vi "AlliGator Phasor Ratio Graph Panel.vi"() -> ()   [LabVIEW 2021, in "AlliGator Phasor Ratio.lvlib"]
uses:
  AlliGator Phasor Ratio.lvlib
  Phasor/Phasor Ratio Type.ctl
  AlliGator Phasor Ratio Graph Ctrl Refnums.ctl
  Globals, Variables, Constants/AlliGator Refnums List.ctl
  Settings/AlliGator Settings List.ctl
  Graphs/XY Graph/XY Graph Event.ctl
  <vilib>/Utility/miscctls.llb/LVPoint32TypeDef.ctl
  Action Engine/AlliGator Q Element.ctl
  Action Engine/AlliGator Q Event.ctl
  Graphs/XY Graph/XY Graph Mouse Click Event Data.ctl
  Graphs/XY Graph/XY Graph Refnum.ctl
  Graphs/XY Graph/New Plot Information.ctl
  Graphs/Plot Scales.ctl
  Graphs/LabVIEW Plot Interpolation.ctl
  Graphs/Plot Point Style.ctl
  Lifetime & Other Parameters/AlliGator Lifetime & Other Parameters Ctrl Refnums.ctl
  Variant/Variant to Data/Variant to Boolean.vi
  Settings/AlliGator Settings+.lvlib
  Variant/Variant to Data/Variant to Data.lvlib
  Notebook/Notebook.lvlib
  Action Engine/AlliGator Action Engine.lvlib
  GUI/GUI.lvlib
  GUI/AlliGator GUI.lvlib
  Error/Error.lvlib
  Graphs/XY Graph/XY Graph Add-Ons.lvlib
  Python Plugins API/AlliGator Python Plugins.lvlib
  Decay Analysis/Decay Processing/AlliGator Decay Processing.lvlib
  Graphs/Graphs.lvlib
  Lifetime & Other Parameters/AlliGator Lifetime & Other Parameters.lvlib
  Utilities/Utilities.lvlib
  Phasor/Phasor.lvlib
panel:
  in  "Pin Button":bool=TRUE
  out "Phasor Ratio Graph TipStrip":string caption="Lifetime Graph TipStrip"
  out "Phasor Ratio Graph":cluster{"X Array":dbl[], "Y Array":dbl[]}[](graph)
  in  "Phasor Ratio Type":T1
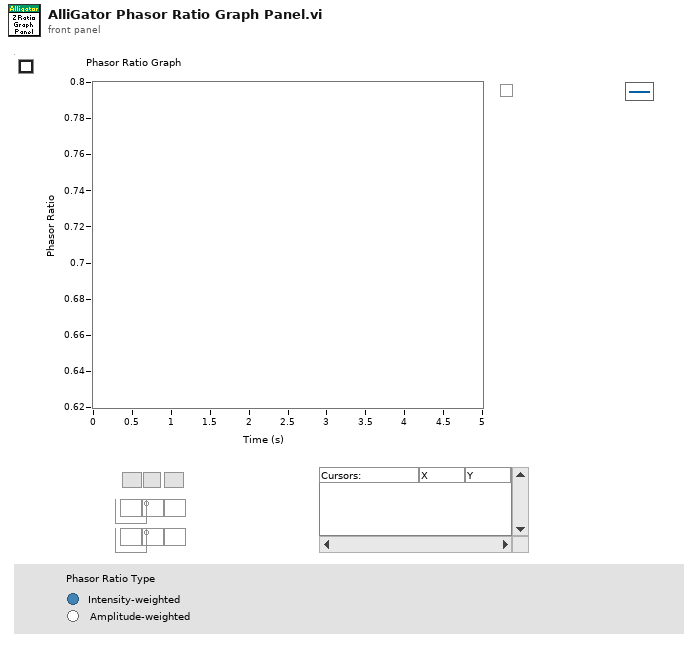
[diagram p1: front panel]
types:
  T1 = typedef "Phasor.lvlib/Phasor Ratio Type.ctl" = enum32{"Intensity-weighted", "Amplitude-weighted"}
  T2 = typedef "AlliGator GUI.lvlib/AlliGator Refnums List.ctl" = enum16{"---------- AlliGator Control Refnums ----------", "AlliGator Tab Control Refnum", "Dataset Ctrl Refnums", "Image Histogram Ctrl Refnums", "Intensity Time Trace Ctrl Refnums", "Decay Graph Ctrl Refnums", "Decay Statistics Graph Ctrl Refnums", "Phasor Graph Ctrl Refnums", "Phasor Ratio Graph Ctrl Refnums", "Phasor Plot Ctrl Refnums", "Lifetime & Other Parameters Ctrl Refnums", "Decay Fit Parameter Map Ctrl Refnums", "Parameter Map Ctrl Refnums", "Other AlliGator Ctrl Refnums", "---------- AlliGator Menu Refnums ----------", "AlliGator Menu", "---------- IO Device ID ----------", "Mouse ID", "Keyboard ID"}
  T3 = typedef "AlliGator Phasor Ratio.lvlib/AlliGator Phasor Ratio Graph Ctrl Refnums.ctl" = cluster{"Phasor Ratio Graph":refnum<vi>}
  T4 = cluster{"Event Registration Refnum":refnum<event-registration>, "Event Registration Refnum":refnum<event-registration>}
  T5 = typedef "AlliGator Settings+.lvlib/AlliGator Settings List.ctl" = enum16{"GUI:Visible Settings Tab", "GUI:Last Run Version", "Source Image:Use Image Histogram for Contrast", "Source Image:Low Count Pixels Rejection Options", "Source Image:High Count Pixels Rejection Options", "Source Image:Use Image Brightness", "Source Image:Blend Overlay with Image Background", "Source Image:Use Fixed ROI Diameter", "Source Image:ROI Diameter", "Source Image:ROI Center Color", "Source Image:Peak Threshold", "Source Image:Intensity Threshold", "Source Image:Image Binning Options", "Source Image:Image Smoothing Options", "Source Image:Image Histogram Active", "Source Image:Invert Binary Mask", "Source Image:Hot Pixel Removal", "Source Image:Overlay Analyzed ROI Center", "Source Image:Auto-Adjust Contrast", "Source Image:Histogram Lower Percentile", "Source Image:Histogram Upper Percentile", "Source Image:Lock ROI with Maps", "Source Image:Save Source Image", "Source Image:Scale Bar Options", "Source Image:Image Resolution (Pixel Size)", "Source Image:Flatfield Correction", "Source Image:Show Dead Left Columns Correction", "Source Image:Dead Left Columns Correction", "Source Image:Image Pre-Processing Operations Order", "Source Image:Overlay ROI Median", "Source Image:Median Overlay Color", "Data Information:Gate Width", "Data Information:Nanotime Gate Separation", "Data Information:Macrotime Gate Separation", "Data Information:Gate Step", "Data Information:# Gates", "Data Information:Gate Image Exposure", "Data Information:Gate Image Integration", "Data Information:Gates to Skip", "Data Information:Gates to Keep", "Data Information:Define Gates to", "Data Information:Channel Name", "Data Information:Available Channel Names", "Data Information:Channel Arithmetic", "Data Information:Background File Subtraction", "Data Information:Background File", "Data Information:Background Scaling Factor", "Data Information:Background Pile-up Correction", "Data Information:Background Pixel Well Capacity", "Data Information:Laser Period", "Data Information:SYNC Period", "Data Information:Pile-up Correction", "Data Information:Pixel Well Capacity", "Data Information:Dataset Scaling Factor", "Fluorescence Decay_Decay Pre-Processing:Reverse Gates", "Fluorescence Decay_Decay Pre-Processing:Verbose Decay Pre-Processing", "Fluorescence Decay_Decay Pre-Processing:Use Decay Pre-Processing", "Fluorescence Decay_Decay Pre-Processing:Background Subtraction", "Fluorescence Decay_Decay Pre-Processing:Background Definition Range", "Fluorescence Decay_Decay Pre-Processing:Baseline Subtraction Method", "Fluorescence Decay_Decay Pre-Processing:Decay Pre-Processing Operations Order", "Fluorescence Decay_Decay Pre-Processing:Smoothing Parameter", "Fluorescence Decay_Decay Pre-Processing:Shift Decay", "Fluorescence Decay_Decay Pre-Processing:Decay Shift Parameters", "Fluorescence Decay_Decay Pre-Processing:Fold Decay", "Fluorescence Decay_Decay Pre-Processing:# Folds", "Fluorescence Decay_Decay Pre-Processing:1-Normalize Decay", "Fluorescence Decay_Decay Pre-Processing:[0-1]-Normalize Decay", "Fluorescence Decay_Decay Pre-Processing:Smoothen Decay", "Fluorescence Decay_Decay Pre-Processing:Extrapolate Decay", "Fluorescence Decay_Decay Pre-Processing:Use Periodicity", "Fluorescence Decay_Decay Pre-Processing:Use Cursors", "Fluorescence Decay_Decay Pre-Processing:Tail Fraction", "Fluorescence Decay_Decay Pre-Processing:Head Fraction", "Fluorescence Decay_Decay Pre-Processing:Additional Points", "Fluorescence Decay_Decay Pre-Processing:Straighten Decay", "Fluorescence Decay_Decay Pre-Processing:Constant Background", "Fluorescence Decay_Decay Pre-Processing:Pixel-Normalize Decay", "Fluorescence Decay_Advanced Analysis:Extract IRF instead of Decay", "Fluorescence Decay_Advanced Analysis:IRF Extraction Options", "Fluorescence Decay_Advanced Analysis:IRF Optimization Options", "Fluorescence Decay_Advanced Analysis:Square Pulse Options", "Fluorescence Decay_Advanced Analysis:IRF Order", "Fluorescence Decay_Advanced Analysis:IRF Time Constants", "Fluorescence Decay_Advanced Analysis:Wavelet Analysis Options", "Fluorescence Decay_Advanced Analysis:Average Lifetime Options", "Fluorescence Decay_Fit Options:Fit Options", "Fluorescence Decay_Fit Options:Use Legacy Fitting Approach", "Fluorescence Decay_Fit Options:Use Data Information Laser Period", "Fluorescence Decay_Fit Parameters:Displayed Fit Parameters", "Fluorescence Decay_Fit Parameters:Fit Parameter Constraints", "Fluorescence Decay_Fit Parameters:Export Tabulated Results", "Fluorescence Decay_Fit Parameters:MLE Baseline Offset Type", "Fluorescence Decay_Fit Parameters:MLE Baseline Offset", "Fluorescence Decay_Fit Parameters:Guess Parameter Names", "Fluorescence Decay_Fit Parameters:Guess Parameter Values", "Fluorescence Decay_Fit Parameters:Guess Parameters Options", "Fluorescence Decay_Fit Parameters:Optimal Offset Selection Criterion", "Fluorescence Decay_Styles:Show Last Decay Only", "Fluorescence Decay_Styles:Decay Graph Color Array", "Fluorescence Decay:Decay Graph Active", "Fluorescence Decay Statistics:Min Peak Value", "Fluorescence Decay Statistics:Reject Low Decay Peak Pixels", "Fluorescence Decay Statistics:Reject High Decay Peak Pixels", "Fluorescence Decay Statistics:Max Peak Value", "Time Traces:Use File Timestamp", "Time Traces:Time Step", "Time Traces:Use Intensity Correction File", "Time Traces:Intensity Correction File", "Phasor Plot:Phasor Plot Smoothing Options", "Phasor Plot:Phasor Plot Size", "Phasor Plot:Phasor Plot Graphics Options", "Phasor Plot:Cumulative Phasor Plot", "Phasor Plot:Use Phasor Brightness", "Phasor Plot:Blend Overlay with Phasor Background", "Phasor Plot:Save Phasor Plot", "Phasor Plot:Show References", "Phasor Plot:Phasor Ratio Decay Range", "Phasor Plot:Exponential Fading", "Phasor Plot:Phasor Ratio Reference Colors", "Phasor Plot:Reference Radius", "Phasor Plot:Show Color Map Vertices", "Phasor Plot:Phasor Plot Active", "Phasor Plot:Phasor Ratio Color Map Type", "Phasor Plot:Phasor Ratio Color Map", "Phasor Plot:Phasor Ratio Display Range", "Phasor Plot:Selected Image ROI(s)", "Phasor Plot:All Image ROIs", "Phasor Plot:Selected Phasor Plot ROI(s)", "Phasor Plot:All Phasor Plot ROIs", "Phasor Plot:Phasor Ratio Color-Coded Quantity", "Phasor Plot:Store Phasor Harmonics", "Phasor Plot:Draw Reference Segment", "Phasor Plot:User-Defined Quantity", "Phasor Plot:Color Scale High Color", "Phasor Plot:Color Scale Low Color", "Phasor Plot:Intensity-weighted Phasor Plot", "Phasor Graph:Phasor Frequency", "Phasor Graph:Phasor Ratio Type", "Phasor Graph:Pixel-level Phasor Computation", "Phasor Graph:Save Phasor Graph", "Phasor Graph:Phasor Graph Active", "Phasor Graph:Phasor SDV Options", "Phasor Graph:Intensity-weighted Phasor Graph", "Phasor Graph:Define Shortest Lifetime as", "Phasor Calibration:Use Backup Calibration if needed", "Phasor Calibration:Backup Calibration Type", "Phasor Calibration:Calibration Type", "Phasor Calibration:Calibration Lifetime", "Phasor Calibration:Calibration Map Algorithm", "Single-Exponential Phasor Locus (SEPL):Gate Parameters", "Single-Exponential Phasor Locus (SEPL):User-defined Gate", "Single-Exponential Phasor Locus (SEPL):User-defined IRF", "Single-Exponential Phasor Locus (SEPL):Phasor Parameters", "Single-Exponential Phasor Locus (SEPL):Decay & IRF Parameters", "Single-Exponential Phasor Locus (SEPL):Display Parameters", "Lifetime Analysis:Decay Analysis Parameters", "Lifetime Analysis:Lifetime Map Active", "Plugins:Python Settings", "Miscellaneous:Verbose Mode", "Miscellaneous:Beep after Script", "Miscellaneous:Saved Image File Format", "Miscellaneous:Exported Gate Image Settings", "Miscellaneous:Include Loading in Timing", "Miscellaneous:Verbose Settings Mode", "Miscellaneous:Histogram Options", "Miscellaneous:Beep on Error", "Miscellaneous:# Logical Processors Used", "Miscellaneous:ROI Description Max Characters", "Miscellaneous:Verbose Error Mode", "Miscellaneous:Transparent Mask Color"}
  T6 = typedef "XY Graph Add-Ons.lvlib/XY Graph Event.ctl" = cluster{"Item Tag":string, "XY Graph Refnum":refnum<vi>, "Coords":T7, "Item Path":string}
  T7 = typedef "LVPoint32TypeDef.ctl" = cluster{"Horizontal":i32, "Vertical":i32}
  T8 = enum16{"0", "1", "2", "3", "4", "5", "6", "7", "8", "9", "A", "B", "C", "D", "E", "F", "G", "H", "I", "J", "K", "L", "M", "N", "O", "P", "Q", "R", "S", "T", "U", "V", "W", "X", "Y", "Z", "F1", "F2", "F3", "F4", "F5", "F6", "F7", "F8", "F9", "F10", "F11", "F12", "F13", "F14", "F15", "ADD", "BACK", "BACKSLASH", "CAPITAL", "COMMA", "DECIMAL", "DELETE", "DIVIDE", "DOWN", "END", "EQUALS", "ESCAPE", "GRAVE (`)", "HOME", "INSERT", "LBRACKET", "LCONTROL", "LEFT", "L ALT", "LSHIFT", "LWIN", "MINUS", "MULTIPLY", "NEXT", "NUMLOCK", "NUMPAD_0", "NUMPAD_1", "NUMPAD_2", "NUMPAD_3", "NUMPAD_4", "NUMPAD_5", "NUMPAD_6", "NUMPAD_7", "NUMPAD_8", "NUMPAD_9", "PAUSE", "PERIOD", "PRIOR (PG UP)", "RBRACKET", "RCONTROL", "RETURN", "RIGHT", "R ALT", "RSHIFT", "RWIN", "SCROLL", "SEMICOLON", "SLASH", "SPACE", "SUBTRACT", "TAB", "UP", "ENTER (num pad)", "' (quote)"}
  T9 = typedef "AlliGator Action Engine.lvlib/AlliGator Q Element.ctl" = cluster{"AlliGator Q Event":T10, "Data":variant}
  T10 = typedef "AlliGator Action Engine.lvlib/AlliGator Q Event.ctl" = enum16{"---- Files ----", "Files:Set Batch Export Files To Save", "Files:Set Dataset Loading & Pre-processing Options", "Files:Check #Frames in Dataset", "Files:Increment Frame Index", "Files:Open Mask Image", "Files:Open White Light Image", "Files:Open Single Dataset", "Files:New Folder of Folders Selected", "Files:Load File (all Types)_Scriptable", "Files:Move Flattened Series to Folders Series", "Files:Select Folder", "Files:Load FLI Dataset", "Files:Load Swiss SPAD 1 Dataset", "Files:Load Swiss SPAD 2 Dataset", "Files:Load .sdt FLI Dataset", "Files:Load .ptu FLI Dataset", "Files:Load .bin FLI Dataset", "Files:Load Single Gate Image Folder", "Files:Load I/m/phi Dataset (deprecated)", "Files:Load Single Image", "Files:Subtract Background File", "Files:Export FLI Dataset", "Files:Load HDF5 FLI Dataset", "Files:Set Destination File Path", "Files:Save Mask Image", "Files:Batch Conversion", "Files:New Folder Selected", "Files:Close FLI Dataset", "Files:Close FLI Dataset Series", "Files:Close White Light Image", "Files:Close Mask Image", "---- FLI Dataset ----", "FLI Dataset:Channel Arithmetic", "FLI Dataset:Export Average Lifetime Map as ASCII", "FLI Dataset:Export User-Defined Quantity Map as ASCII", "FLI Dataset:Python Function FLI Dataset Event", "FLI Dataset:ROI Analysis", "FLI Dataset:Tilted Logistic Square Gated IRF Characteristics Map", "FLI Dataset:Logistic Square Gated IRF Characteristics Map", "FLI Dataset:Square Gated IRF Characteristics Map", "FLI Dataset:Multi-ROI Single-Pixel Phasor Analysis", "FLI Dataset:Multi-ROI Single-Pixel NLSF Analysis", "FLI Dataset:All ROIs IRF Extraction", "FLI Dataset:All ROIs Decay Fit Non-Interactive (Fast + Individual IRF)", "FLI Dataset:All ROIs Phasor Analysis", "FLI Dataset:All ROIs Decay Fit", "FLI Dataset:Fluorescence Decay Statistics", "FLI Dataset:Update Decay Statistics Graph", "FLI Dataset:Get Decay from ROI", "FLI Dataset:All ROIs Average Lifetimes", "FLI Dataset:Save/Load Local IRFs", "FLI Dataset:Clear Local IRFs", "FLI Dataset:Phasor Calibration Maps (# Gates Series) Script", "FLI Dataset:Calibrated Phasor Map Series", "---- FLI Dataset Series ----", "FLI Dataset Series:Sum All Datasets in Series", "FLI Dataset Series:Add Dataset to Accumulated Dataset", "FLI Dataset Series:Display Accumulated Dataset", "FLI Dataset Series:Clear Dataset Series Sum", "FLI Dataset Series:Time-Series Analysis (NLSF)", "FLI Dataset Series:Time-Series Analysis (Phasor)", "---- Image ----", "Image:Update Image Profile Plots", "Image:Image Histogram Cursor Move", "Image:Image Histogram", "Image:Image Contrast", "Image:Set Image Histogram Cursor Move Flag", "Image:Clear Image Overlay", "Image:Use ROI as Search Area", "Image:Set ROI Diameter", "Image:Save Image Data as TIFF", "Image:Save Displayed Image with Overlay", "Image:Save Image Overlay Only", "Image:Save Image as Hot Pixel Mask", "Image:Change Source Image Color Palette", "Image:Copy Image to Clipboard", "Image:Source Image ROI Selection", "Image:Delete All ROIs", "Image:Delete All Unselected ROIs", "Image:Delete ROI", "Image:Merge All ROIs", "Image:Store ROI", "Image:Source Image ROI Storage", "Image:Export ROI Description to Notebook", "Image:Save ROI", "Image:Load ROI", "Image:Paste ROI Definition", "Image:Clear ROI", "Image:Identify ROIs in Mask Image", "Image:Create Complementary ROI", "Image:Create Contour ROI", "Image:Create ROI(s) from Pixels with Peak above Min_Scriptable", "Image:Create ROI(s) from Pixels with Intensity above Min_Scriptable", "Image:Compute ROI Statistics", "Image:Delete ROI(s) based on ROI Characteristics", "Image:Create ROI Grid", "Image:ROI to Individual Pixel ROIs", "Image:Python Function Source Image Event", "Image:Show Phasor Calibration Map ROI Centers", "Image:Convert ROI to Mask Image", "Image:Mouse Move", "Image:Mouse Up", "Image:Set Source Image Mouse Move Flag", "Image:Add Scale Bar Overlay", "Image:Delete Existing ROIs Option", "Image:Overlay ROI Median", "Image:Check Current ROI", "Image:Update True Pixel Value", "Image:Use ROI", "---- Decay ----", "Decay:Clear IRF/Reference Plot", "Decay:Add Decay to Graph", "Decay:Smoothen Plot", "Decay:Smoothen Plot Tail", "Decay:Average Selected Plots", "Decay:Extract IRF", "Decay:Optimal IRF Extraction", "Decay:Threshold IRF", "Decay:Fit to Model IRF", "Decay:Fit IRF to Square Gate", "Decay:Fit IRF to Logistic Square Gate", "Decay:Fit IRF to Tilted Logistic Square Gate", "Decay:Create Bounding Cursors Set", "Decay:Export Bounding Cursors Definition to Notebook", "Decay:Denoise Plot", "Decay:Compute Cumulative Function", "Decay:Use as Reference Decay", "Decay:Show Reference Decay/IRF", "Decay:Extrapolate Decay", "Decay:Create Head & Tail Bounding Cursors", "Decay:Store Cursor-defined Head & Tail Fractions", "Decay:Rebin Plot", "Decay:1-Normalize Decay", "Decay:[0-1]-Normalize Plot", "Decay:Straighten Decay", "Decay:Shift Decay", "Decay:Fold Decay", "Decay:Fit Decay", "Decay:Global Fit of Selected Decays", "Decay:Post Global Fit Script", "Decay:Add Global Fit Parameters to Graph", "Decay:Add Decay Parameter(s) to Plot (Graph)", "Decay:Export Decay to Phasor Graph", "Decay:Compute Average Lifetime", "Decay:Plot Convolution", "Decay:Graph Tip Strip Update", "---- Decay Statistics ----", "Decay Statistics:Tip Strip Update", "---- Intensity Time Trace ----", "Intensity Time Trace:Use File Timestamp", "Intensity Time Trace:Load Intensity Corrections File", "Intensity Time Trace:Clear Intensity Corrections File", "Intensity Time Trace:Tip Strip Update", "---- Phasor Plot ----", "Phasor Plot:Build Phasor Plot", "Phasor Plot:Change Phasor Plot Color Palette", "Phasor Plot:Adjust Phasor Plot Display Range", "Phasor Plot:Highlight Image ROI in Phasor Plot", "Phasor Plot:Save Phasor Plot Image with Overlay", "Phasor Plot:Export Complex Phasor Map", "Phasor Plot:Export Phasor Ratio Map", "Phasor Plot:Export Average Lifetime Map", "Phasor Plot:Compute Phase Lifetime Histogram", "Phasor Plot:Compute Phasor Ratio Histogram", "Phasor Plot:Compute Phase Lifetime vs Intensity Scatter Plot", "Phasor Plot:Weber 2-Component Decomposition", "Phasor Plot:Update Phasor Color Map Vertices", "Phasor Plot:Clear Phasor Overlay", "Phasor Plot:Use Segment Extremities as References", "Phasor Plot:Use UC/Segment Intersections as References", "Phasor Plot:Use UC/Principal Axis Intersections as References", "Phasor Plot:Use UC/Linear Fit Intersections as References", "Phasor Plot:Update Phasor Plot Reference", "Phasor Plot:Show Local Phasor Info in Phasor Plot", "Phasor Plot:Update Phasor Plot State", "Phasor Plot:Phasor Plot ROI Storage", "Phasor Plot:Phasor Plot ROI Selection", "Phasor Plot:Python Function Phasor Plot Event", "Phasor Plot:Overlay Phasor ROI, Ratio or Map in Source Image", "Phasor Plot:Compute Decay of Selected Phasors", "Phasor Plot:Phasor at Image Pixel", "Phasor Plot:Mouse Move", "Phasor Plot:Mouse Up", "Phasor Plot:Display Range Mouse Move", "Phasor Plot:Set Mouse Move Flag", "Phasor Plot:Update True Phasor Plot Value", "---- Phasor Graph ----", "Phasor Graph:Get Phasor Value", "Phasor Graph:Create New Phasor Plot Dialog", "Phasor Graph:Update Last Phasor Value", "Phasor Graph:Update Phasor (m, phi)", "Phasor Graph:Remove Single Phasor from Plot", "Phasor Graph:Add Single Phasor to Plot", "Phasor Graph:Remove Phasor Plot", "Phasor Graph:Remove Selected Phasor Plots", "Phasor Graph:Clear Phasor Data", "Phasor Graph:Clear Phasor Graph", "Phasor Graph:Cursor Move", "Phasor Graph:Draw Cursor Connecting Line", "Phasor Graph:Clear Cursor Connecting Line", "Phasor Graph:Find UC Intersection", "Phasor Graph:Use UC/Cursor-Defined Line Intersections", "Phasor Graph:Use Selected Plots Fitted Line/UC Intersections", "Phasor Graph:Use Selected Plots Principal Axis/UC Intersections", "Phasor Graph:Show Single Phasor", "Phasor Graph:Save Single Phasor Plot", "Phasor Graph:Save All Phasor Plots", "Phasor Graph:Load Phasor Plot(s)", "Phasor Graph:Phasor Multiplication", "Phasor Graph:Compute Average Phasor", "Phasor Graph:Compute Multiple Average Phasors (Selected Plots)", "Phasor Graph:Export Single Phasor Plot Phase Lifetimes", "Phasor Graph:Parameter 2 vs Parameter 1 Scatter Plot", "Phasor Graph:Use Cursor n Location", "Phasor Graph:Set Reference n to Current Phase Lifetime Value", "Phasor Graph:Set Reference n to Lifetime Value", "Phasor Graph:Set Cursor n Location", "Phasor Graph:Save Phasor Graph Image", "Phasor Graph:Update SEPL Plot", "Phasor Graph:Export Single Phasor Plot Data", "Phasor Graph:Export Selected Phasor Plots Data", "Phasor Graph:Python Function Phasor Graph Event", "Phasor Graph:Tip Strip Update", "---- Calibration ----", "Calibration:Set Calibration Type", "Calibration:Load/Save Phasor Calibration", "Calibration:Load/Save Phasor Calibration Series", "Calibration:Load/Save Phasor Calibration Map", "Calibration:Use as Calibration", "Calibration:Compute Optimal Calibration from Phasor References", "Calibration:Clear Phasor Calibration", "Calibration:Single Phasor Calibration Information", "Calibration:Use as Calibration Series", "Calibration:Use as Calibration Map", "Calibration:Clear Calibration Series", "Calibration:Phasor Calibration Series Information", "Calibration:Clear Calibration Map", "Calibration:Phasor Calibration Map Information", "Calibration:Apply Phasor Calibration", "Calibration:Update Single Plot Calibration", "Calibration:Update Multiple Plots Calibration", "Calibration:Clear Single Plot Calibration", "Calibration:Clear All Plots Calibrations", "Calibration:Clear Plot(s) Calibration(s)?", "---- Phasor Ratio ----", "Phasor Ratio:Clear Reference n", "Phasor Ratio:Toggle Selected Plot(s)  Lock to Reference 1", "Phasor Ratio:Use as Reference n", "Phasor Ratio:Send Reference n to Notebook", "Phasor Ratio:Toggle Selected Plot(s)  Lock to Reference 2", "Phasor Ratio:Compute Phasor Ratio at Mouse Location", "Phasor Ratio:Compute Phasor Plot's Average Phasor Ratio", "Phasor Ratio:Compute Time-Series Phasor Ratios", "Phasor Ratio:Fit Line to Phasor Ratio Plot", "Phasor Ratio:Save References", "Phasor Ratio:Load References", "Phasor Ratio:Update Phasor Reference 1", "Phasor Ratio:Update Phasor Reference 2", "Phasor Ratio:Move Cursor n to Reference n", "Phasor Ratio:Use as Phasor Reference 1 Lifetime", "Phasor Ratio:Use as Phasor Reference 2 Lifetime", "Phasor Ratio:Export Phasor Ratio Map as ASCII", "Phasor Ratio:Tip Strip Update", "---- Lifetime & Other Parameters Graph ----", "Lifetime:Compute Sliced Mean, SDV and CV Plots", "Lifetime:Plot Decay Shifts", "Lifetime:Plot Histogram", "---- Decay Fit Parameter Map ----", "Decay Fit Parameter Map:Export ROI NLSF Data as ASCII", "Decay Fit Parameter Map:Set Decay Fit Parameter Map Selection", "Decay Fit Parameter Map:Build Decay Fit Parameter Map", "Decay Fit Parameter Map:Change Decay Fit Parameter Map Color Palette", "Decay Fit Parameter Map:Export Decay Fit Parameter Map Data as ASCII", "Decay Fit Parameter Map:Export All Decay Fit Parameter Maps Data as ASCII", "Decay Fit Parameter Map:Selected Parameter Scatterplot", "Decay Fit Parameter Map:Parameter 2 vs Parameter 1 Scatterplot", "Decay Fit Parameter Map:Save Decay Fit Parameter Map Image", "Decay Fit Parameter Map:Save-Load IRFs & Fit Data", "Decay Fit Parameter Map:Update Local Decay Plots", "Decay Fit Parameter Map:Python Function Decay Fit Parameters Map Event", "Decay Fit Parameter Map:Overlay Decay Fit Parameter Map in Source Image", "Decay Fit Parameter Map:Selected Parameter vs Intensity Scatterplot", "Decay Fit Parameter Map:Mouse Up", "Decay Fit Parameter Map:Mouse Move", "Decay Fit Parameter Map:Display Range Mouse Move", "Decay Fit Parameter Map:Change Map Resolution", "Decay Fit Parameter Map:Variance Significance Maps", "Decay Fit Parameter Map:Fit Result Constraints Window", "Decay Fit Parameter Map:Use ROI", "---- Parameter Map ----", "Parameter Map:Export ROI Parameters Data as ASCII", "Parameter Map:Add Parameter Map Set", "Parameter Map:Delete Parameter Map Set", "Parameter Map:Update Parameter List", "Parameter Map:Build Parameter Map", "Parameter Map:Change Parameter Map Color Palette", "Parameter Map:Export Parameter Map Data as ASCII", "Parameter Map:Export All Parameter Maps Data as ASCII", "Parameter Map:Selected Parameter Scatterplot", "Parameter Map:Parameter 2 vs Parameter 1 Scatterplot", "Parameter Map:Selected Parameter vs Intensity Scatterplot", "Parameter Map:Save Parameter Map Image", "Parameter Map:Save-Load IRFs & Parameter Maps (TODO)", "Parameter Map:Set Parameter Map Selection", "Parameter Map:Python Function Parameter Map Event", "Parameter Map:Overlay Parameter Map in Source Image", "Parameter Map:Update Local Decay Plots", "Parameter Map:Mouse Up", "Parameter Map:Mouse Move", "Parameter Map:Display Range Mouse Move", "Parameter Map:Use ROI", "---- Generic Graph ----", "Generic Graph:Generic XY Graph Event", "Generic Graph:Python Function XY Graph Event", "Generic Graph:New Plot", "Generic Graph:Save Plot", "Generic Graph:XY Plot Histogram", "Generic Graph:Set XY Graph Plot Name", "Generic Graph:Set Last Cursor Style", "Generic Graph:Tip Strip Update", "---- GUI ----", "GUI:Start Script", "GUI:Type of Displayed Image Changed", "GUI:Gate Image Slide Changed", "GUI:Show Busy Icon", "GUI:Show Busy Icon & Abort Button", "GUI:Hide Busy Icon", "GUI:Hide Busy Icon & Abort Button", "GUI:Abort", "GUI:End Script", "GUI:Start Timing", "GUI:End Timing", "GUI:Set State Indicator", "GUI:Send Parameters JSON Strings to Clipboard", "GUI:Set Gate Step", "GUI:Idle", "GUI:Initialization", "GUI:Quit", "GUI:Increment Dataset Index", "GUI:Set Dataset Index to -1", "GUI:Time Series Slider Moved", "GUI:Time Series Slider Changed", "GUI:Toggle Playback or Loop", "GUI:Playback Script", "GUI:Set Phasor Frequency", "GUI:Open Window", "GUI:Start Test Script", "GUI:End Test Script", "GUI:Set Verbose Mode", "GUI:Set Verbose Settings Mode", "GUI:Initialize Python Session", "DEBUG"}
  T11 = typedef "XY Graph Add-Ons.lvlib/XY Graph Mouse Click Event Data.ctl" = cluster{"Multiplot XY Graph":T12, "Mouse Coordinates":T7}
  T12 = typedef "XY Graph Add-Ons.lvlib/XY Graph Refnum.ctl" = refnum<vi>
  T13 = typedef "AlliGator Lifetime & Other Parameters.lvlib/AlliGator Lifetime & Other Parameters Ctrl Refnums.ctl" = cluster{"Lifetime Graph":refnum<vi>}
  T14 = enum16{"0", "1", "2", "3", "4", "5", "6", "7", "8", "9", "A", "B", "C", "D", "E", "F", "G", "H", "I", "J", "K", "L", "M", "N", "O", "P", "Q", "R", "S", "T", "U", "V", "W", "X", "Y", "Z", "F1", "F2", "F3", "F4", "F5", "F6", "F7", "F8", "F9", "F10", "F11", "F12", "F13", "F14", "F15", "ADD", "BACK", "BACKSLASH", "CAPITAL", "COMMA", "DECIMAL", "DELETE", "DIVIDE", "DOWN", "END", "EQUALS", "ESCAPE", "GRAVE (`)", "HOME", "INSERT", "LBRACKET", "LCONTROL", "LEFT", "L ALT", "LSHIFT", "LWIN", "MINUS", "MULTIPLY", "NEXT", "NUMLOCK", "NUMPAD_0", "NUMPAD_1", "NUMPAD_2", "NUMPAD_3", "NUMPAD_4", "NUMPAD_5", "NUMPAD_6", "NUMPAD_7", "NUMPAD_8", "NUMPAD_9", "PAUSE", "PERIOD", "PRIOR (PG UP)", "RBRACKET", "RCONTROL", "RETURN", "RIGHT", "R ALT", "RSHIFT", "RWIN", "SCROLL", "SEMICOLON", "SLASH", "SPACE", "SUBTRACT", "TAB", "UP", "ENTER (num pad)", "' (quote)"}[]
  T15 = typedef "XY Graph Add-Ons.lvlib/New Plot Information.ctl" = cluster{"Multiplot XY Graph":refnum<vi>, "Plot Name":string, "Plot Scales":T16, "Plot Interpolation":T17, "Point Style":T18, "Plot Color":u32, "Plot Metadata":variant}
  T16 = typedef "XY Graph Add-Ons.lvlib/Plot Scales.ctl" = cluster{"X Scale":u32, "Y Scale":u32}
  T17 = typedef "Graphs.lvlib/LabVIEW Plot Interpolation.ctl" = enum16{"Point (.)", "Stepwise Right (--.)", "Line + Point (\\. /)", "Stepwise Left (.--)", "Stepwise Centered (-.-)", "Stepwise Vertical (|.|)", "Line (-)", "Use Previous Plot's Style"}
  T18 = typedef "Graphs.lvlib/Plot Point Style.ctl" = enum16{"not defined", "None", "Empty Circle", "Filled Circle", "Thick Circle", "Dotted Circle", "Empty Square", "Filled Square", "Thick Square", "Dotted Square", "Small Filled Square", "Dot", "Cross", "Tiny Cross", "Large X", "Small x", "Diamond", "Small Empty Square"}
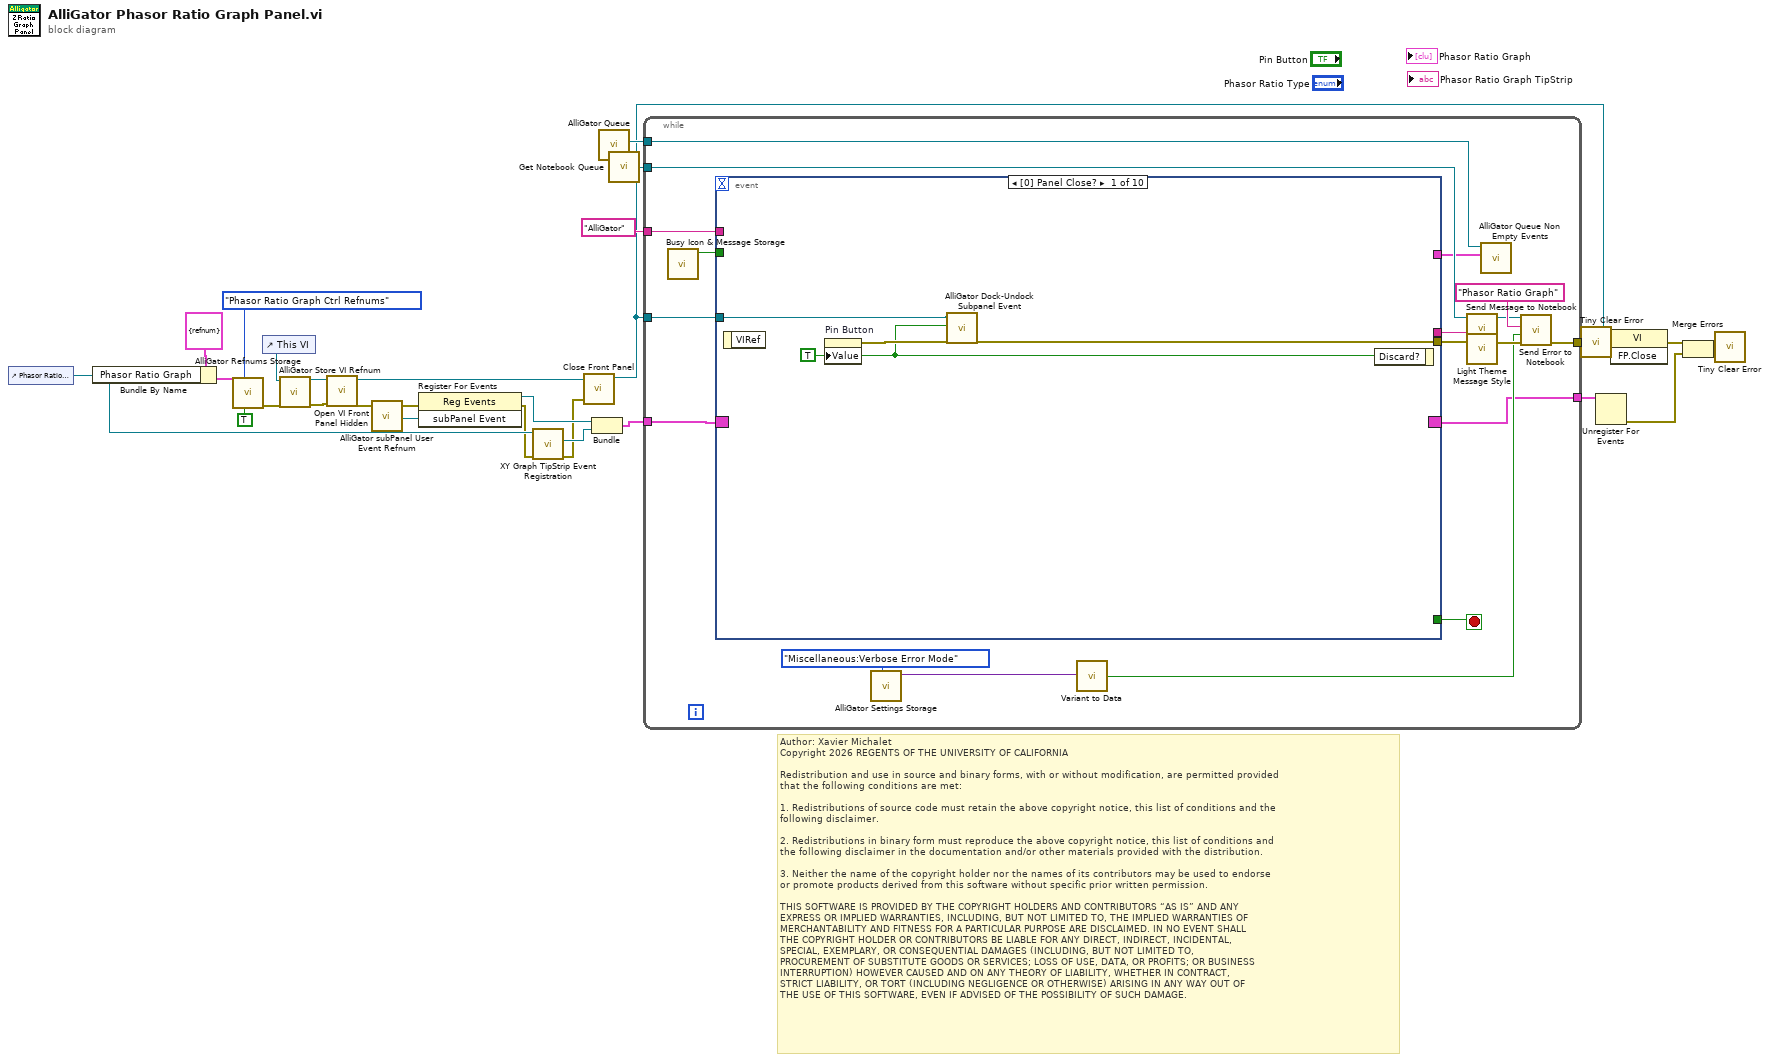
[diagram p0: block diagram]
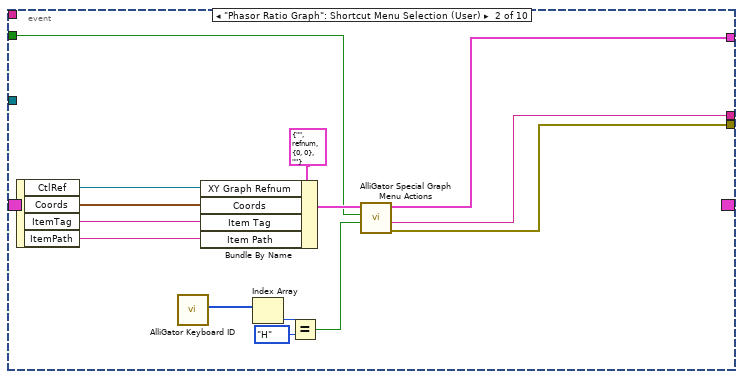
[diagram p2: hidden frame]
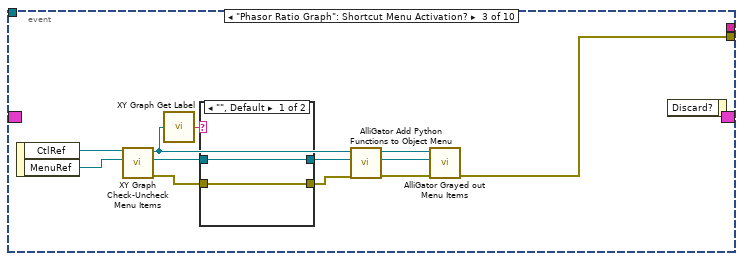
[diagram p3: hidden frame]
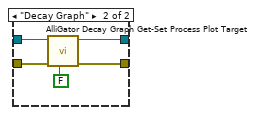
[diagram p4: hidden frame]
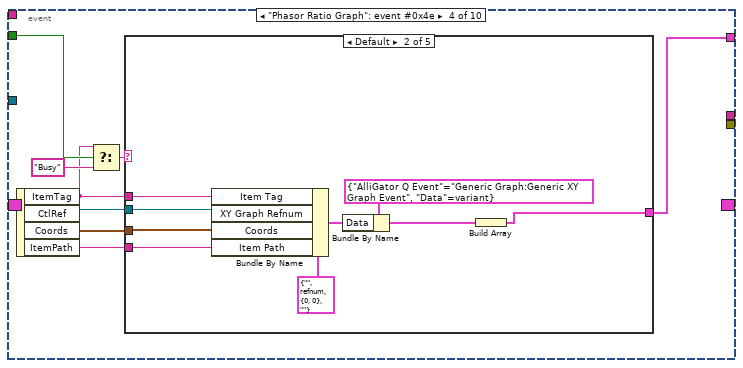
[diagram p5: hidden frame]
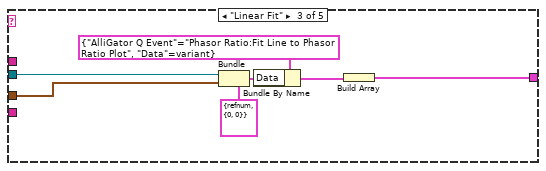
[diagram p7: hidden frame]
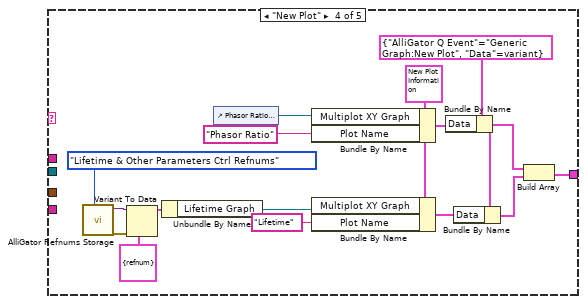
[diagram p8: hidden frame]
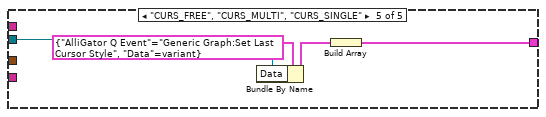
[diagram p9: hidden frame]
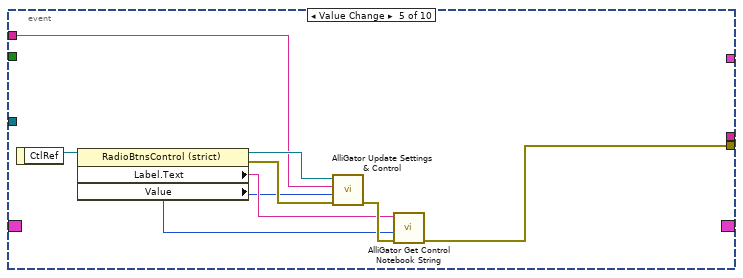
[diagram p10: hidden frame]
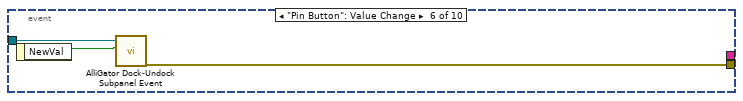
[diagram p11: hidden frame]
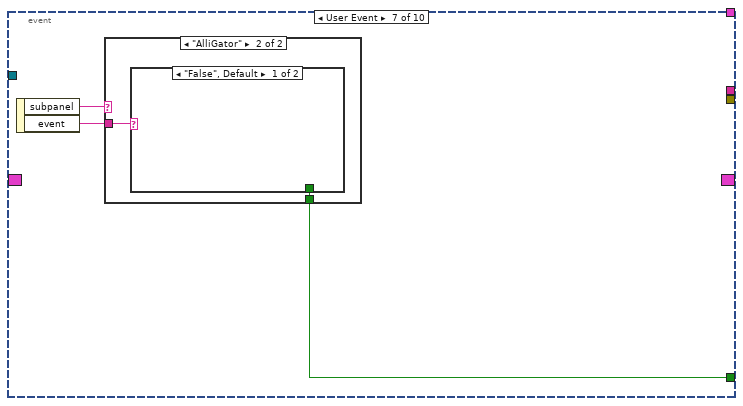
[diagram p12: hidden frame]
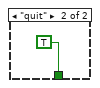
[diagram p14: hidden frame]
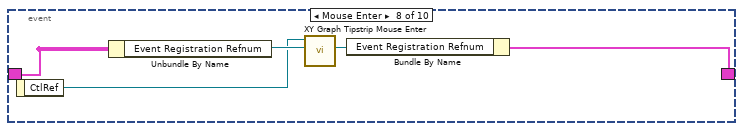
[diagram p15: hidden frame]
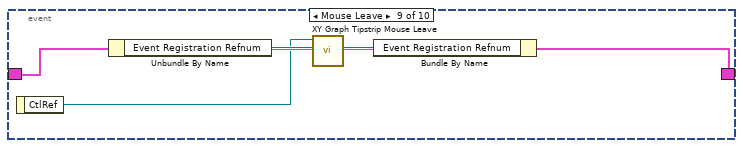
[diagram p16: hidden frame]
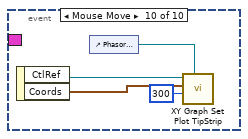
[diagram p17: hidden frame]
diagram:
  # "Author: Xavier Michalet\nCopyright 2026 REGENTS OF THE UNIVERSITY OF CALIFORNIA\n\nRedistribution and use in source and binary forms, with or without modification, are permitted provided\nthat the following conditions are met:\n\n1. Redistributions of source code must retain the above copyright notice, this list of conditions and the\nfollowing disclaimer.\n\n2. Redistributions in binary form must reproduce the above copyright notice, this list of conditions and\nthe following disclaimer in the documentation and/or other materials provided with the distribution.\n\n3. Neither the name of the copyright holder nor the names of its contributors may be used to endorse \nor promote products derived from this software without specific prior written permission.\n\nTHIS SOFTWARE IS PROVIDED BY THE COPYRIGHT HOLDERS AND CONTRIBUTORS “AS IS” AND ANY \nEXPRESS OR IMPLIED WARRANTIES, INCLUDING, BUT NOT LIMITED TO, THE IMPLIED WARRANTIES OF\nMERCHANTABILITY AND FITNESS FOR A PARTICULAR PURPOSE ARE DISCLAIMED. IN NO EVENT SHALL\nTHE COPYRIGHT HOLDER OR CONTRIBUTORS BE LIABLE FOR ANY DIRECT, INDIRECT, INCIDENTAL, \nSPECIAL, EXEMPLARY, OR CONSEQUENTIAL DAMAGES (INCLUDING, BUT NOT LIMITED TO, \nPROCUREMENT OF SUBSTITUTE GOODS OR SERVICES; LOSS OF USE, DATA, OR PROFITS; OR BUSINESS\nINTERRUPTION) HOWEVER CAUSED AND ON ANY THEORY OF LIABILITY, WHETHER IN CONTRACT, \nSTRICT LIABILITY, OR TORT (INCLUDING NEGLIGENCE OR OTHERWISE) ARISING IN ANY WAY OUT OF\nTHE USE OF THIS SOFTWARE, EVEN IF ADVISED OF THE POSSIBILITY OF SUCH DAMAGE."
  n1 = control-ref of="Phasor Ratio Graph"() -> (w15:refnum<vi>)
  n2 = Bundle By Name(cluster=T3 {"Phasor Ratio Graph"=refnum} ("Phasor Ratio Graph Ctrl Refnums"), "Phasor Ratio Graph"=w15) -> (w16:T3)
  n3 = call "AlliGator Refnums Storage.vi"("Get(F)/Set"=TRUE, "AlliGator Refnum List"=AlliGator_Refnums_List."Phasor Ratio Graph Ctrl Refnums", "Data in"=w16) -> ("Error Out"=w4:errorcluster)  [unwired: 7 in, 1 out]
  n4 = control-ref of="This VI"() -> (w1:refnum<vi>)
  n5 = call "AlliGator Store VI Refnum.vi"("error in (no error)"=w4, "VI Refnum"=w1) -> ("error out"=w3:errorcluster, "VI Refnum (dup)"=w2:refnum<vi>)  [unwired: 7 in, 1 out]
  n6 = call "Open VI Front Panel Hidden.vi"("error in"=w3, "VI in"=w2) -> ("error out"=w9:errorcluster, "VI out"=w7:refnum<vi>)  [unwired: 8 in]
  n7 = call "AlliGator subPanel User Event Refnum.vi"() -> ("subPanel Event"=w24:refnum<user-event>)  [unwired: 9 in]
  n8 = register-events(error in=w9, w24) -> (reference out=w23:refnum<event-registration>, error out=w8:errorcluster)  [unwired: 1 in]
  n9 = call "XY Graph TipStrip Event Registration.vi"("error in (no error)"=w8, "XY Graph Refnum"=w15) -> ("error out"=w6:errorcluster, "Event Registration Refnum"=w13:refnum<event-registration>)  [unwired: 7 in, 1 out]
  n10 = call "Close Front Panel.vi"("error in (no error)"=w6, "VI in"=w7) -> ("VI out"=w5:refnum<vi>)  [unwired: 8 in, 1 out]
  n11 = Bundle("Event Registration Refnum"=w23, "Event Registration Refnum"=w13) -> (w14:T4)  [unwired: 1 in]
  n12 = call "AlliGator Queue.vi"() -> ("AlliGator Q"=w26:refnum<queue>)  [unwired: 8 in, 1 out]
  n13 = call "Get Notebook Queue.vi"() -> ("Notebook Queue"=w27:refnum<queue>)  [unwired: 9 in]
  n14 = while {
    tunnel: w27 -> [w38]
    tunnel: w26 -> [w35]
    tunnel: "AlliGator" ("Sender") -> [w33]
    tunnel: w5 -> [w31]
    tunnel: w14 -> [w30]
    tunnel: [w29] -> w22
    tunnel: [w28] -> w21
    stop <- w45 stop-if-true
    n15 = call "Busy Icon & Message Storage.vi"() -> ("Busy Icon Status (F = busy)"=w32:bool)  [unwired: 9 in, 2 out]
    n16 = event shown="[0] Panel Close?" {
      selector: w30 -> [_ _ _ _ _ _ _ w146 w151 _]
      dyn-events: [_ _ _ _ _ _ _ w144 w149 _] -> w29
      timeout: _ -> [_ _ _ _ _ _ _ _ _ _]
      tunnel: [w48 w50 w64 _ w127 w135 _ _ _ _] -> w39
      tunnel: [_ _ _ _ _ _ w138 _ _ _] -> w45
      tunnel: [_ w51 _ _ _ _ _ _ _ _] -> w36
      tunnel: [_ w52 _ w89 _ _ _ _ _ _] -> w34
      tunnel: w32 -> [_ w57 _ w88 _ _ _ _ _ _]
      tunnel: w33 -> [_ _ _ _ w130 _ _ _ _ _]
      tunnel: w31 -> [w47 _ _ _ _ w137 _ _ _ _]
      event Panel Close? {
        w46 = TRUE ("Pin Button")
        n17 = event-data() -> ()  [unwired: 1 in, 1 out]
        n18 = property on="Pin Button" class="Bool (strict)"("Value"=w46) -> (error out=w49:errorcluster)  [unwired: 2 in, 1 out]
        n19 = call "AlliGator Dock-Undock Subpanel Event.vi"("Error In"=w49, "Dock?"=w46, "VI in"=w47) -> ("Error Out"=w48:errorcluster)  [unwired: 8 in]
        n20 = event-data("Discard?"=w46) -> ()  [unwired: 1 in, 1 out]
      }
      event "Phasor Ratio Graph": Shortcut Menu Selection (User) {
        n21 = event-data() -> ("CtlRef"=w53:refnum<vi>, "Coords"=w56:T7, "ItemTag"=w54:string, "ItemPath"=w55:string)  [unwired: 1 in]
        n22 = call "AlliGator Keyboard ID.vi"() -> ("keys pressed"=w63:T14)  [unwired: 9 in, 2 out]
        n23 = Bundle By Name(cluster=T6 {"Item Tag"="", "XY Graph Refnum"=refnum, "Coords"={"Horizontal"=0, "Vertical"=0}, "Item Path"=""} ("XY Graph Event"), "XY Graph Refnum"=w53, "Coords"=w56, "Item Tag"=w54, "Item Path"=w55) -> (w61:T6)
        n24 = Index Array(array=w63) -> (element=w58:T8)  [unwired: 1 in]
        n25 = Equal?(x=w58, y=T8."H" ("element")) -> (x = y?=w62:bool)
        n26 = call "AlliGator Special Graph Menu Actions.vi"("Help?"=w62, "Animated Busy Icon"=w57, "XY Graph Event"=w61) -> ("Error Out"=w50:errorcluster, "Message"=w51:string, "AlliGator Actions"=w52:T9[])  [unwired: 6 in]
      }
      event "Phasor Ratio Graph": Shortcut Menu Activation? {
        n27 = event-data() -> ("CtlRef"=w66:refnum<vi>, "MenuRef"=w65:refnum<k9>)  [unwired: 1 in]
        n28 = call "XY Graph Check-Uncheck Menu Items.vi"("Menu in"=w65, "XY Graph Refnum"=w66) -> ("Error Out (dup)"=w75:errorcluster, "Menu out"=w70:refnum<k9>, "XY Graph Refnum dup"=w68:T12)  [unwired: 6 in, 1 out]
        n29 = call "XY Graph Get Label.vi"("XYGraph"=w68) -> ("Graph Label"=w67:string)  [unwired: 8 in]
        n30 = case shown="\"\", Default" w67 {
          tunnel: w75 -> [w76 w82]
          tunnel: [w76 w81] -> w71
          tunnel: w70 -> [w77 w80]
          tunnel: [w77 w79] -> w69
          frame "", Default {
          }
          frame "Decay Graph" {
            n31 = call "AlliGator Decay Graph Get-Set Process Plot Target.vi"("Get (F)/Set"=FALSE, "Error In"=w82, "Menu"=w80) -> ("Error Out (dup)"=w81:errorcluster, "Menu"=w79:refnum<k9>)  [unwired: 6 in, 1 out]
          }
        }
        n32 = call "AlliGator Add Python Functions to Object Menu.vi"("error in (no error)"=w71, "Menu in"=w69, "Object Refnum"=w68) -> ("error out"=w74:errorcluster, "Menu out"=w73:refnum<k9>, "Object Refnum dup"=w72:refnum<vi>)  [unwired: 6 in]
        n33 = call "AlliGator Grayed out Menu Items.vi"("error in (no error)"=w74, "Menu in"=w73, "Object Refnum"=w72) -> ("error out"=w64:errorcluster)  [unwired: 7 in, 1 out]
        n34 = event-data() -> ()  [unwired: 2 in, 1 out]
      }
      event "Phasor Ratio Graph": event #0x4e {
        n35 = event-data() -> ("ItemTag"=w84:string, "CtlRef"=w90:refnum<vi>, "Coords"=w86:T7, "ItemPath"=w83:string)  [unwired: 1 in]
        n36 = Select(t=w84, s=w88, f="Busy") -> (s? t:f=w85:string)
        n37 = case shown="Default" w85 {
          tunnel: w90 -> [_ w94 w102 _ w123]
          tunnel: [_ w91 w100 w116 w125] -> w89
          tunnel: w86 -> [_ w93 w101 _ _]
          tunnel: w84 -> [_ w95 _ _ _]
          tunnel: w83 -> [_ w92 _ _ _]
          frame "", "Busy" {
          }
          frame Default {
            n38 = Bundle By Name(cluster=T6 {"Item Tag"="", "XY Graph Refnum"=refnum, "Coords"={"Horizontal"=0, "Vertical"=0}, "Item Path"=""} ("XY Graph Event"), "Item Tag"=w95, "XY Graph Refnum"=w94, "Coords"=w93, "Item Path"=w92) -> (w97:T6)
            n39 = Bundle By Name(cluster=T9 {"AlliGator Q Event"=enum."Generic Graph:Generic XY Graph Event", "Data"=variant} ("element"), "Data"=w97) -> (w99:T9)
            n40 = Build Array(w99) -> (w91:T9[])
          }
          frame "Linear Fit" {
            n41 = Bundle(cluster=T11 {"Multiplot XY Graph"=refnum, "Mouse Coordinates"={"Horizontal"=0, "Vertical"=0}} ("Mouse Click Event Data"), "Multiplot XY Graph"=w102, "Mouse Coordinates"=w101) -> (w104:T11)
            n42 = Bundle By Name(cluster=T9 {"AlliGator Q Event"=enum."Phasor Ratio:Fit Line to Phasor Ratio Plot", "Data"=variant} ("Time-Gated Phasor Q Element"), "Data"=w104) -> (w103:T9)
            n43 = Build Array(w103) -> (w100:T9[])
          }
          frame "New Plot" {
            w118 = T15 {"Multiplot XY Graph"=refnum, "Plot Name"="", "Plot Scales"={"X Scale"=0, "Y Scale"=0}, "Plot Interpolation"=enum."Use Previous Plot's Style", "Point Style"=enum."not defined", "Plot Color"=15781887, "Plot Metadata"=variant} ("New Plot Information")
            n44 = call "AlliGator Refnums Storage.vi"("AlliGator Refnum List"=AlliGator_Refnums_List."Lifetime & Other Parameters Ctrl Refnums") -> ("Error Out"=w111:errorcluster, "Data out"=w112:variant)  [unwired: 9 in]
            n45 = Variant To Data(error in=w111, type=T13 {"Lifetime Graph"=refnum} ("Lifetime & Other Parameters Graph Ctrl Refnums"), Variant=w112) -> (data=w109:T13)  [unwired: 1 out]
            n46 = Unbundle By Name(w109) -> ("Lifetime Graph"=w108:refnum<vi>)
            n47 = control-ref of="Phasor Ratio Graph"() -> (w119:refnum<vi>)
            n48 = Bundle By Name(cluster=w118, "Multiplot XY Graph"=w119, "Plot Name"="Phasor Ratio") -> (w122:T15)
            n49 = Bundle By Name(cluster=w118, "Multiplot XY Graph"=w108, "Plot Name"="Lifetime") -> (w117:T15)
            n50 = Bundle By Name(cluster=T9 {"AlliGator Q Event"=enum."Generic Graph:New Plot", "Data"=variant} ("Time-Gated Phasor Q Element"), "Data"=w122) -> (w114:T9)
            n51 = Bundle By Name(cluster=w114, "Data"=w117) -> (w115:T9)
            n52 = Build Array(w114, w115) -> (w116:T9[])
          }
          frame "CURS_FREE", "CURS_MULTI", "CURS_SINGLE" {
            n53 = Bundle By Name(cluster=T9 {"AlliGator Q Event"=enum."Generic Graph:Set Last Cursor Style", "Data"=variant} ("AlliGator Actions"), "Data"=w123) -> (w124:T9)
            n54 = Build Array(w124) -> (w125:T9[])
          }
        }
      }
      event Value Change {
        n55 = event-data() -> ("CtlRef"=w133:refnum<vi>)  [unwired: 1 in]
        n56 = property class="RadioBtnsControl (strict)"(reference=w133) -> (reference out=w132:refnum<vi>, error out=w131:errorcluster, "Label.Text"=w129:string, "Value"=w128:T1)  [unwired: 1 in]
        n57 = call "AlliGator Update Settings & Control.vi"("Error In"=w131, "Value"=w128, "Sender"=w130, "CtlRef"=w132) -> ("Error Out"=w134:errorcluster)  [unwired: 7 in]
        n58 = call "AlliGator Get Control Notebook String.vi"("error in (no error)"=w134, "Value"=w128, "Control Label"=w129) -> ("error out"=w127:errorcluster)  [unwired: 7 in, 1 out]
      }
      event "Pin Button": Value Change {
        n59 = event-data() -> ("NewVal"=w136:bool)  [unwired: 1 in]
        n60 = call "AlliGator Dock-Undock Subpanel Event.vi"("Dock?"=w136, "VI in"=w137) -> ("Error Out"=w135:errorcluster)  [unwired: 9 in]
      }
      event User Event {
        n61 = event-data() -> ("subpanel"=w140:string, "event"=w139:string)  [unwired: 1 in]
        n62 = case shown="\"AlliGator\"" w140 {
          tunnel: w139 -> [_ w142]
          tunnel: [_ w141] -> w138
          frame "False", Default {
          }
          frame "AlliGator" {
            n63 = case shown="\"False\", Default" w142 {
              tunnel: [_ TRUE] -> w141
              frame "False", Default {
              }
              frame "quit" {
              }
            }
          }
        }
      }
      event Mouse Enter {
        n64 = event-data() -> ("CtlRef"=w145:refnum<vi>)  [unwired: 1 in]
        n65 = Unbundle By Name(w146) -> ("Event Registration Refnum"=w148:refnum<event-registration>)
        n66 = call "XY Graph Tipstrip Mouse Enter.vi"("Event Registration Refnum"=w148, "XY Graph Refnum"=w145) -> ("Event Registration Refnum"=w147:refnum<event-registration>)  [unwired: 8 in, 1 out]
        n67 = Bundle By Name(cluster=w146, "Event Registration Refnum"=w147) -> (w144:T4)
      }
      event Mouse Leave {
        n68 = event-data() -> ("CtlRef"=w150:refnum<vi>)  [unwired: 1 in]
        n69 = Unbundle By Name(w151) -> ("Event Registration Refnum"=w152:refnum<event-registration>)
        n70 = call "XY Graph Tipstrip Mouse Leave.vi"("Event Registration Refnum"=w152, "XY Graph Refnum"=w150) -> ("Event Registration Refnum"=w153:refnum<event-registration>)  [unwired: 8 in, 1 out]
        n71 = Bundle By Name(cluster=w151, "Event Registration Refnum"=w153) -> (w149:T4)
      }
      event Mouse Move {
        n72 = event-data() -> ("CtlRef"=w156:refnum<vi>, "Coords"=w155:T7)  [unwired: 1 in]
        n73 = control-ref of="Phasor Ratio Graph TipStrip"() -> (w154:refnum<vi>)
        n74 = call "XY Graph Set Plot TipStrip.vi"("TipStrip Refnum"=w154, "Max Length (200)"=300, "Coords"=w155, "XY Graph Refnum"=w156) -> ()  [unwired: 5 in, 3 out]
      }
    }
    n75 = call "AlliGator Settings Storage.vi"("AlliGator Settings List"=AlliGator_Settings_List."Miscellaneous:Verbose Error Mode") -> ("Variant Data out"=w44:variant)  [unwired: 9 in, 1 out]
    n76 = call-poly "Variant to Data.vi"("Variant"=w44) -> ("Value"=w37:bool)  [unwired: 8 in]
    n77 = call "Send Message to Notebook.vi"("Error In"=w39, "Text"=w36, "Notebook Queue"=w38) -> ("Error Out"=w41:errorcluster, "Notebook Queue"=w40:refnum<queue>)  [unwired: 5 in]
    n78 = call "Light Theme Message Style.vi"() -> ()  [unwired: 1 out]
    n79 = call "AlliGator Queue Non Empty Events.vi"("Actions"=w34, "AlliGator Q"=w35) -> ()  [unwired: 9 in, 1 out]
    n80 = call "Send Error to Notebook.vi"("error in (no error)"=w41, "Verbose Error Messages (T)"=w37, "State Machine Case Error Source"="Phasor Ratio Graph", "Notebook Q"=w40) -> ("Error Out"=w28:errorcluster)  [unwired: 7 in]
  }
  n81 = call "Tiny Clear Error.vi"("Error In"=w21) -> ("no Error Out"=w20:errorcluster)  [unwired: 8 in]
  n82 = Unregister For Events(event registration refnum=w22) -> (error out=w11:errorcluster)  [unwired: 1 in]
  n83 = invoke class="VI" method="FP.Close"(reference=w5, error in=w20) -> (error out=w12:errorcluster)  [unwired: 1 in, 2 out]
  n84 = Merge Errors(w12, w11) -> (w10:errorcluster)
  n85 = call "Tiny Clear Error.vi"("Error In"=w10) -> ()  [unwired: 8 in, 1 out]
